vi "Add Text Input.vi"(7 "title":string, 8 "error in (no error)":errorcluster, 9 "placeHolderContent":string, 10 "id":string, 11 "reference":refnum<k24>) -> (0 "error out":errorcluster, 3 "reference out":refnum<k24>)   [LabVIEW 2026, in "ToastNotification.lvlib" / "Toast Native.lvlib"]
doc: "Native AddInputTextBox call using id, placeHolderContent and title. Borrow the builder and return its reference alias. id becomes the key of the submitted UserInput value. The placeholder is a visual hint, not a default reply. Does not expose DefaultInput, close the builder or register a callback."
uses:
  Toast Native.lvlib
  C:/Users/loicw/Documents/LabVIEW/ToastNotifications/Sources/bins/Microsoft.Toolkit.Uwp.Notifications.dll
  bins/Microsoft.Toolkit.Uwp.Notifications.dll
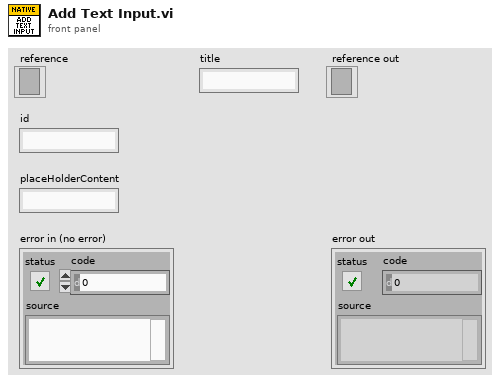
[diagram p1: front panel]
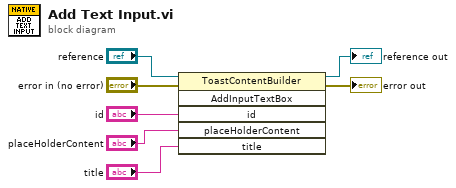
[diagram p0: block diagram]
diagram:
  n1 = invoke class="ToastContentBuilder" method="AddInputTextBox"(reference="reference", error in="error in (no error)", "id"="id", "placeHolderContent"="placeHolderContent", "title"="title") -> (reference out=→"reference out":refnum<k24>, error out=→"error out":errorcluster)  [unwired: 1 in, 4 out]
